vi "RT_VFD_Adapter.vi"(8 "error in (no error)":errorcluster={"status"=FALSE, "code"=0, "source"="\"\""}, 10 "status query":string, 11 "Speed request":string) -> (0 "error out":errorcluster={"status"=FALSE, "code"=0, "source"="\"\""}, 2 "status ok":bool, 3 "Applied ACK":string)   [LabVIEW 2026]
doc: "INTENT: Implement selected VFD protocol. LOGIC: Encode protocol/PROFINET/Modbus write, read fault/speed feedback and correlate command; separate transport failure."
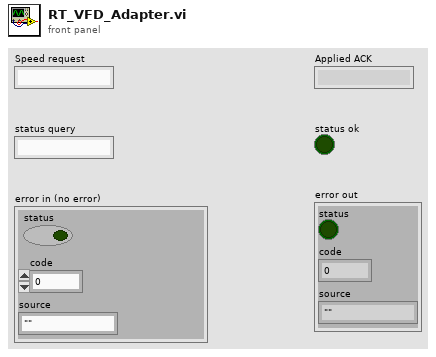
[diagram p1: front panel]
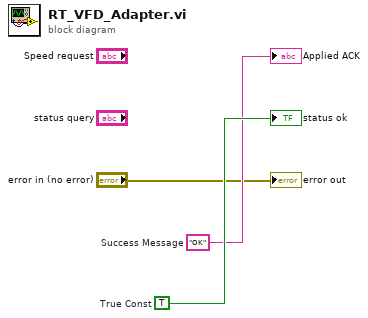
[diagram p0: block diagram]
diagram:
  w3 = TRUE  # True Const
  w2 = "OK"  # Success Message
  "Applied ACK" <- w2
  "status ok" <- w3
  "error out" <- "error in (no error)"
